vi "Cast.vi"(4 "Number of Shifts":i32, 6 "Lookup Table":sgl[](array[numeric]), 7 "Method":T1 items=["Use Bit Depth", "Shift", "Use Lookup Table"], 8 "error in":errorcluster, 9 "Image Type":T2, 10 "Image Dst Reference In":T3, 11 "Image Src Reference In":T3) -> (0 "error out":errorcluster, 3 "Image Dst Reference Out":T3)   [LabVIEW 2020, in "OpenLvVision_Image.lvlib" / "Management.lvlib"]
doc: "Converts the image's pixel data type."
uses:
  Management.lvlib
  TypeDef/Image.ctl
  TypeDef/ImageType.ctl
  TypeDef/CastMethode.ctl
  DataAccess/DataAccess.lvlib
  DLLs/OLV_VisionCore_AVX2_X86.dll
  DLLs/OLV_VisionCore_AVX2_X64.dll
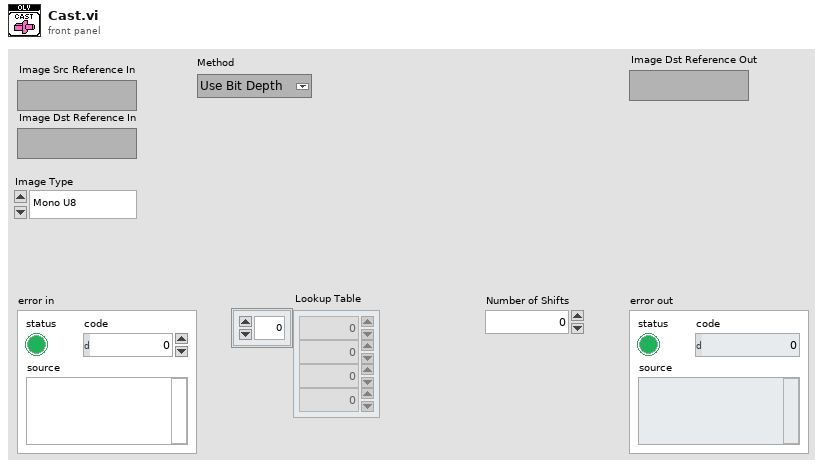
[diagram p1: front panel]
types:
  T1 = typedef "OpenLvVision_Image.lvlib/Management.lvlib/CastMethode.ctl" = u32
  T2 = typedef "OpenLvVision_Image.lvlib/Management.lvlib/ImageType.ctl" = enum16{"Mono U8", "Mono U16", "Mono I16", "Mono SGL", "Color U32", "Color U64", "Complex CSG"}
  T3 = typedef "OpenLvVision_Image.lvlib/Management.lvlib/Image.ctl" = refnum<image>
  T4 = typedef "OpenLvVision_Image.lvlib/DataAccess.lvlib/ImagePointer.ctl" = cluster{"ImagePointer":u64, "BorderSize":i32, "LineWidth":i32, "Width":i32, "Height":i32, "ImageFormat":T2}
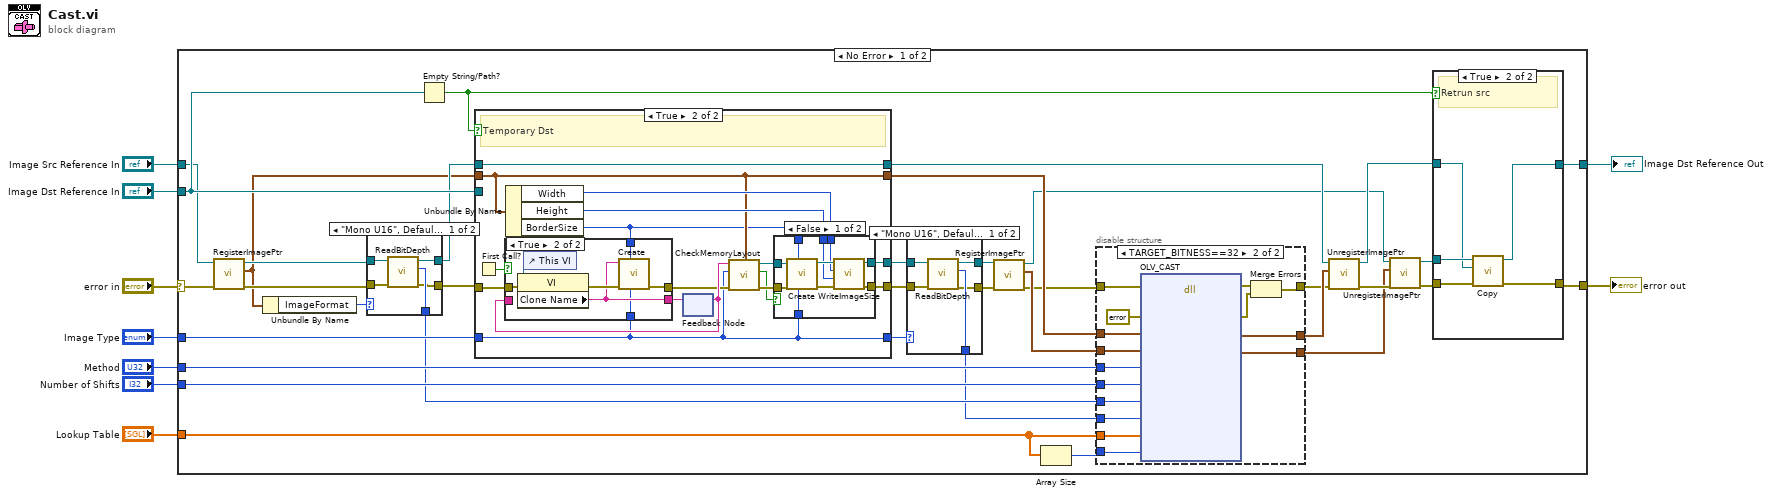
[diagram p0: block diagram]
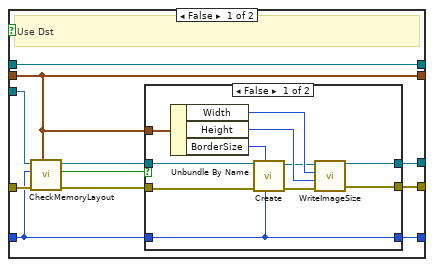
[diagram p3: hidden frame]
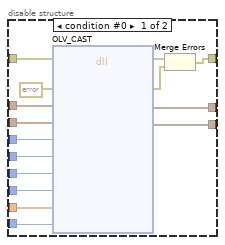
[diagram p8: hidden frame]
diagram:
  n1 = case shown="No Error" "error in" {
    selector: "error in" -> [w18 w159]
    tunnel: [w26 w159] -> w8
    tunnel: "Image Dst Reference In" -> [w34 _]
    tunnel: "Image Src Reference In" -> [w19 w160]
    tunnel: "Image Type" -> [w33 _]
    tunnel: "Lookup Table" -> [w44 _]
    tunnel: "Number of Shifts" -> [w43 _]
    tunnel: "Method" -> [w42 _]
    tunnel: [w36 w160] -> w1
    frame No Error {
      n2 = call "RegisterImagePtr.vi"("error in"=w18, "Image Reference In"=w19) -> ("error out"=w17:errorcluster, "ImagePointer"=w11:T4, "Image Reference Out"=w13:T3)  [unwired: 7 in]
      n3 = Unbundle By Name(w11) -> ("ImageFormat"=w10:T2)
      n4 = case shown="\"Mono U16\", Default" w10 {
        tunnel: w17 -> [w50 w51]
        tunnel: w13 -> [w49 w52]
        tunnel: [w48 w52] -> w12
        tunnel: [w47 _] -> w15
        tunnel: [w46 w51] -> w16
        frame "Mono U16", Default {
          n5 = call "ReadBitDepth.vi"("error in"=w50, "Image Reference In"=w49) -> ("error out"=w46:errorcluster, "BitDepth"=w47:u32, "Image Reference Out"=w48:T3)  [unwired: 7 in]
        }
        frame "Mono U8", "Color U32" {
        }
      }
      n6 = Empty String/Path?(string/path=w34) -> (empty?=w29:bool)
      n7 = case shown="True" w29 {
        tunnel: w16 -> [w62 w88]
        tunnel: [w57 w93] -> w24
        tunnel: w34 -> [w61 _]
        tunnel: w12 -> [w63 w91]
        tunnel: w33 -> [w54 w79]
        tunnel: [w56 w92] -> w23
        tunnel: [w63 w91] -> w32
        tunnel: w11 -> [w55 w80]
        tunnel: [w55 w80] -> w31
        tunnel: [w53 w79] -> w20
        frame False {
          # "Use Dst"
          n8 = call "CheckMemoryLayout.vi"("SrcPointer"=w55, "error in"=w62, "Format"=w54, "DstImage Reference"=w61) -> ("error out"=w60:errorcluster, "Same"=w59:bool, "DstImage Reference"=w58:T3)  [unwired: 5 in]
          n9 = case shown="False" w59 {
            tunnel: w60 -> [w73 w76]
            tunnel: w58 -> [w74 w77]
            tunnel: [w71 w76] -> w57
            tunnel: [w70 w77] -> w56
            tunnel: w54 -> [w64 w75]
            tunnel: w55 -> [w69 _]
            tunnel: [w64 w75] -> w53
            frame False {
              n10 = Unbundle By Name(w69) -> ("Width"=w66:i32, "Height"=w67:i32, "BorderSize"=w68:i32)
              n11 = call "Create.vi"("Image Type"=w64, "Border"=w68, "error in"=w73, "Image Name"=w74) -> ("error out"=w72:errorcluster, "Image Reference Out"=w65:T3)  [unwired: 6 in]
              n12 = call "WriteImageSize.vi"("error in"=w72, "Height"=w67, "Width"=w66, "Image Reference In"=w65) -> ("error out"=w71:errorcluster, "Image Reference Out"=w70:T3)  [unwired: 6 in]
            }
            frame True {
            }
          }
        }
        frame True {
          # "Temporary Dst"
          n13 = First Call?() -> (First Call?: T/F=w87:bool)
          n14 = Unbundle By Name(w80) -> ("Width"=w90:i32, "Height"=w89:i32, "BorderSize"=w78:i32)
          n15 = feedback #1() -> (w85:string)  [unwired: 1 in]
          n16 = case shown="True" w87 {
            tunnel: w88 -> [w107 w114]
            tunnel: [w107 w111] -> w84
            tunnel: [w106 w110] -> w86
            tunnel: w85 -> [w106 _]
            tunnel: w79 -> [_ w109]
            tunnel: w78 -> [_ w108]
            frame False {
            }
            frame True {
              n17 = control-ref of="This VI"() -> (w113:refnum<vi>)
              n18 = property class="VI"(reference=w113, error in=w114) -> (error out=w112:errorcluster, "Clone Name"=w110:string)  [unwired: 1 out]
              n19 = call "Create.vi"("Image Type"=w109, "Border"=w108, "error in"=w112, "Image Name"=w110) -> ("error out"=w111:errorcluster)  [unwired: 6 in, 1 out]
            }
          }
          n20 = feedback-in #1(w86) -> ()
          n21 = call "CheckMemoryLayout.vi"("SrcPointer"=w80, "error in"=w84, "Format"=w79, "DstImage Reference"=w85) -> ("error out"=w83:errorcluster, "Same"=w81:bool, "DstImage Reference"=w82:T3)  [unwired: 5 in]
          n22 = case shown="False" w81 {
            tunnel: [w102 w104] -> w93
            tunnel: w79 -> [w101 _]
            tunnel: [w99 w105] -> w92
            tunnel: w90 -> [w98 _]
            tunnel: w89 -> [w97 _]
            tunnel: w78 -> [w96 _]
            tunnel: w83 -> [w95 w104]
            tunnel: w82 -> [w94 w105]
            frame False {
              n23 = call "Create.vi"("Image Type"=w101, "Border"=w96, "error in"=w95, "Image Name"=w94) -> ("error out"=w103:errorcluster, "Image Reference Out"=w100:T3)  [unwired: 6 in]
              n24 = call "WriteImageSize.vi"("error in"=w103, "Height"=w97, "Width"=w98, "Image Reference In"=w100) -> ("error out"=w102:errorcluster, "Image Reference Out"=w99:T3)  [unwired: 6 in]
            }
            frame True {
            }
          }
        }
      }
      n25 = case shown="\"Mono U16\", Default" w20 {
        tunnel: w24 -> [w119 w120]
        tunnel: w23 -> [w118 w121]
        tunnel: [w117 w121] -> w22
        tunnel: [w116 _] -> w14
        tunnel: [w115 w120] -> w21
        frame "Mono U16", Default {
          n26 = call "ReadBitDepth.vi"("error in"=w119, "Image Reference In"=w118) -> ("error out"=w115:errorcluster, "BitDepth"=w116:u32, "Image Reference Out"=w117:T3)  [unwired: 7 in]
        }
        frame "Mono U8", "Color U32" {
        }
      }
      n27 = call "RegisterImagePtr.vi"("error in"=w21, "Image Reference In"=w22) -> ("error out"=w25:errorcluster, "ImagePointer"=w35:T4, "Image Reference Out"=w30:T3)  [unwired: 7 in]
      n28 = Array Size(array=w44) -> (size(s)=w45:i32)
      n29 = disable-structure shown="TARGET_BITNESS==32" {
        disable-tunnel: w45 -> [w136 w151]
        disable-tunnel: w44 -> [w135 w150]
        disable-tunnel: w43 -> [w134 w149]
        disable-tunnel: w42 -> [w133 w148]
        disable-tunnel: [w124 w140] -> w28
        disable-tunnel: [w132 w147] -> w40
        disable-tunnel: [w131 w146] -> w39
        disable-tunnel: w25 -> [w130 w145]
        disable-tunnel: w35 -> [w129 w144]
        disable-tunnel: w31 -> [w128 w143]
        disable-tunnel: w15 -> [w123 w138]
        disable-tunnel: w14 -> [w122 w137]
        frame condition #0 {
          n30 = dll-call lib="C:/Users/lukas/Downloads/OpenLvVision_Image/SourceCode/DLLs/OLV_VisionCore_AVX2_X64.dll" fn="OLV_CAST"(error in=w130, "Error"=errorcluster {"status"=FALSE, "code"=0, "source"=""} ("error out"), "SrcImageInfo"=w128, "DstImageInfo"=w129, "Methode"=w133, "NumberOfShifts"=w134, "bitdepthSrc"=w123, "bitdepthDst"=w122, "LookupTable"=w135, "LookupTableSize"=w136) -> (error out=w126:errorcluster, "Error"=w125:errorcluster, "SrcImageInfo"=w132:T4, "DstImageInfo"=w131:T4)  [unwired: 9 in, 1 out]
          n31 = Merge Errors(w126, w125) -> (w124:errorcluster)
        }
        frame condition #1 (active) {
          n32 = dll-call lib="C:/Users/lukas/Downloads/OpenLvVision_Image/SourceCode/DLLs/OLV_VisionCore_AVX2_X86.dll" fn="OLV_CAST"(error in=w145, "Error"=errorcluster {"status"=FALSE, "code"=0, "source"=""} ("error out"), "SrcImageInfo"=w143, "DstImageInfo"=w144, "Methode"=w148, "NumberOfShifts"=w149, "bitdepthSrc"=w138, "bitdepthDst"=w137, "LookupTable"=w150, "LookupTableSize"=w151) -> (error out=w141:errorcluster, "Error"=w139:errorcluster, "SrcImageInfo"=w147:T4, "DstImageInfo"=w146:T4)  [unwired: 9 in, 1 out]
          n33 = Merge Errors(w141, w139) -> (w140:errorcluster)
        }
      }
      n34 = call "UnregisterImagePtr.vi"("error in"=w28, "ImagePointer"=w40, "Image Reference In"=w32) -> ("error out"=w41:errorcluster, "Image Reference Out"=w37:T3)  [unwired: 7 in]
      n35 = call "UnregisterImagePtr.vi"("error in"=w41, "ImagePointer"=w39, "Image Reference In"=w30) -> ("error out"=w27:errorcluster, "Image Reference Out"=w38:T3)  [unwired: 7 in]
      n36 = case shown="True" w29 {
        tunnel: w27 -> [w152 w158]
        tunnel: w38 -> [w153 w156]
        tunnel: w37 -> [_ w155]
        tunnel: [w153 w157] -> w36
        tunnel: [w152 w154] -> w26
        frame False {
          # "Return Dst"
        }
        frame True {
          # "Retrun src"
          n37 = call "Copy.vi"("error in"=w158, "Image Dst Reference In"=w155, "Image Src Reference In"=w156) -> ("error out"=w154:errorcluster, "Image Dst Reference Out"=w157:T3)  [unwired: 7 in]
        }
      }
    }
    frame Error {
    }
  }
  "error out" <- w8
  "Image Dst Reference Out" <- w1
